vi "Stream Length.vi"(8 "error in (no error)":errorcluster, 11 "MCP SSE Response in":refnum<class "MCP SSE Response.lvclass">) -> (0 "error out":errorcluster, 2 "Stream Length":i64, 3 "MCP SSE Response out":refnum<class "MCP SSE Response.lvclass">)   [LabVIEW 2020, in "MCP Server.lvlib" / "MCP SSE Response.lvclass"]
doc: "Returns -1 (unknown length), so the IG HTTP Server streams this response with chunked transfer encoding and keeps calling Next Segment until it reports Last?."
uses:
  MCP SSE Response.lvclass
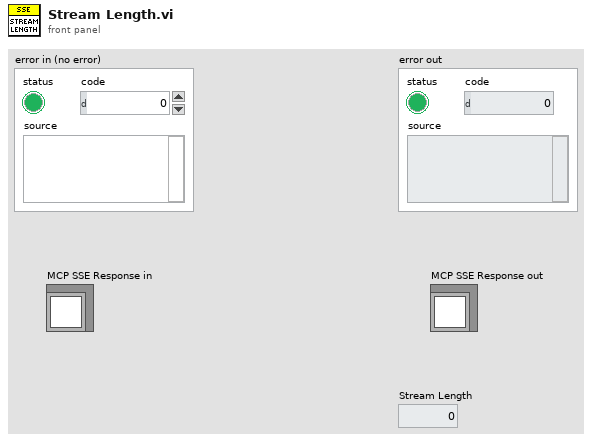
[diagram p1: front panel]
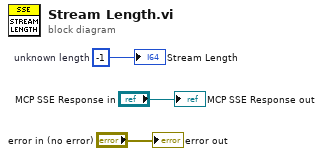
[diagram p0: block diagram]
diagram:
  w1 = i64 -1  # unknown length
  "error out" <- "error in (no error)"
  "MCP SSE Response out" <- "MCP SSE Response in"
  "Stream Length" <- w1
